vi "Convert gRPC UTC Timestamp to String.vi"(11 "access_expires_at":i64) -> (3 "date/time string":string)   [LabVIEW 2020]
doc: "Convert timestamp received through gRPC to a string."
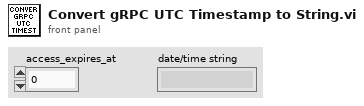
[diagram p1: front panel]
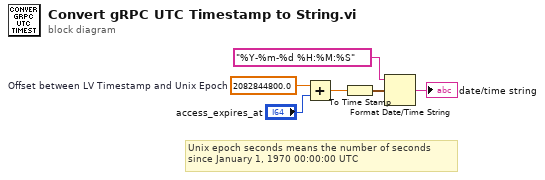
[diagram p0: block diagram]
diagram:
  w3 = 2082844800.0  # Offset between LV Timestamp and Unix Epoch
  # "Unix epoch seconds means the number of seconds\nsince January 1, 1970 00:00:00 UTC"
  n1 = Add(x=w3, y="access_expires_at") -> (x+y=w2:dbl)
  n2 = To Time Stamp(1:w2) -> (0:w1:timestamp)
  n3 = Format Date/Time String(time format string (%c)="%Y-%m-%d %H:%M:%S", seconds (now)=w1) -> (date/time string=→"date/time string":string)  [unwired: 1 in]
